vi "Read Configuration to gRPC.vi"(8 "error in (no error)":errorcluster, 11 "CIFPlugin in":refnum<class "CAN_Reader_CANsub_Plugin.lvclass">) -> (0 "error out":errorcluster, 2 "Configuration":T1={"Common"={"Period (s)"=0.001, "Offset (us)"=0, "Priority"=100, "Processor"=-2, "External Clock"={"ClockID"=0, "Clock Name"="", "Publish Clock"=FALSE, "Convert Data Timestamps"=FALSE, "Plugin Timing Source"=FALSE}}, "RX Interface"="CAN2", "Port Configuration"={"Mode"=enum."CAN FD", "Baud Rate"=500000, "Temination On"=TRUE, "Subordinate"=FALSE, "Echo TX"=FALSE, "FD Config"={"FD Baud Rate"=2000000, "ISO Mode"=TRUE, "BRS Enabled"=TRUE}}, "Timeout (ms)"=100, "Frames to read"=100, "Filter"={"Allow List (ID)"=[], "Deny List (ID)"=[]}} {"Filter"."Deny List (ID)" format="%.0x"; "Filter"."Allow List (ID)" format="%.0x"; "Port Configuration"."FD Config"."FD Baud Rate" format="%.0p"; "Port Configuration"."Baud Rate" format="%.0p"; "Common"."Period (s)" format="%#_13g"}, 3 "CIFPlugin out":refnum<class "CAN_Reader_CANsub_Plugin.lvclass">)   [LabVIEW 2021, in "CAN_Reader_CANsub_Plugin.lvclass"]
doc: "Updates to the configuration will not be automatically updated in the custom gRPC loop. To get the latest configuration the DVR used to pass configuration data from the core gRPC loop to the main loop can be read directly."
uses:
  CAN_Reader_CANsub_Plugin.lvclass
  CAN_Reader_CANsub_Plugin.lvclass/CAN_Reader_CANsub_Plugin.ctl
  <vilib>/CIF Foundation/CIF Core/CIFCore/Class/CIFCorePlugin.lvclass
  C:/Program Files/National Instruments/LabVIEW 2021/vi.lib/CIF Foundation/CIF Core/CIFCore/Class/CIFCorePlugin.lvclass
  D:/dev/Plugins/CAN_Reader_CANsub/Class/CAN_Reader_CANsub_Plugin.lvclass
  <vilib>/CIF Foundation/CIF Core/CIFCore/Common/Typedef/External Clock Config.ctl
  <vilib>/CIF Foundation/CIF Core/CIFCore/Common/CIFCoreCommon.lvlib
  <vilib>/CIF Foundation/CIF Core/CIFCore/Common/Typedef/Common Plugin Configuration.ctl
  Common/Typedef/Configuration.ctl
  Common/CAN_Reader_CANsub_Common.lvlib
  <vilib>/CIF Foundation/CIF CAN RW Core/typedef/CAN Mode.ctl
  <vilib>/CIF Foundation/CIF CAN RW Core/CAN_RW_CORE.lvclass
  <vilib>/CIF Foundation/CIF CAN RW Core/typedef/FD Config.ctl
  <vilib>/CIF Foundation/CIF CAN RW Core/typedef/CAN Port Configuration.ctl
  <vilib>/CIF Foundation/CIF CAN RW Core/typedef/CAN Filter.ctl
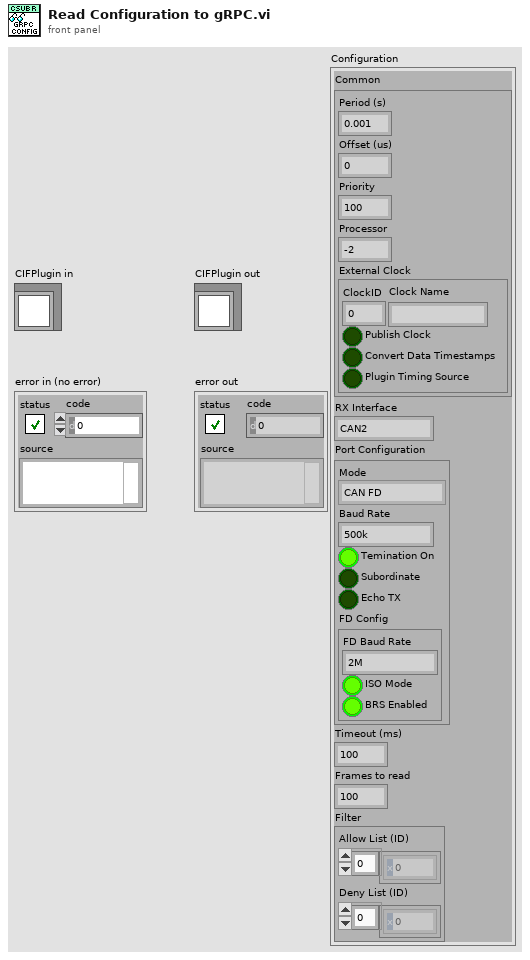
[diagram p1: front panel]
types:
  T1 = typedef "CAN_Reader_CANsub_Common.lvlib/Configuration.ctl" = cluster{"Common":T2, "RX Interface":string, "Port Configuration":T4, "Timeout (ms)":i32, "Frames to read":i32, "Filter":T7}
  T2 = typedef "CIFCoreCommon.lvlib/Common Plugin Configuration.ctl" = cluster{"Period (s)":dbl, "Offset (us)":i32, "Priority":i32, "Processor":i32, "External Clock":T3}
  T3 = typedef "CIFCoreCommon.lvlib/External Clock Config.ctl" = cluster{"ClockID":u8, "Clock Name":string, "Publish Clock":bool, "Convert Data Timestamps":bool, "Plugin Timing Source":bool}
  T4 = typedef "CAN_RW_CORE.lvclass/CAN Port Configuration.ctl" = cluster{"Mode":T5, "Baud Rate":u64, "Temination On":bool, "Subordinate":bool, "Echo TX":bool, "FD Config":T6}
  T5 = typedef "CAN_RW_CORE.lvclass/CAN Mode.ctl" = enum16{"CAN 2.0", "CAN FD"}
  T6 = typedef "CAN_RW_CORE.lvclass/FD Config.ctl" = cluster{"FD Baud Rate":u64, "ISO Mode":bool, "BRS Enabled":bool}
  T7 = typedef "CAN_RW_CORE.lvclass/CAN Filter.ctl" = cluster{"Allow List (ID)":u32[], "Deny List (ID)":u32[]}
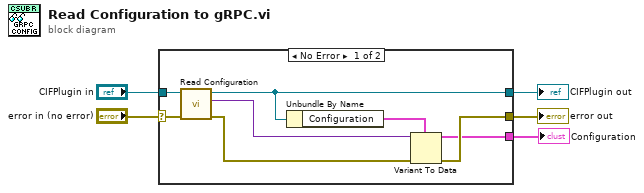
[diagram p0: block diagram]
diagram:
  n1 = case shown="No Error" "error in (no error)" {
    selector: "error in (no error)" -> [w12 w14]
    tunnel: "CIFPlugin in" -> [w13 w15]
    tunnel: [w7 w15] -> w2
    tunnel: [w8 w14] -> w4
    tunnel: [w6 _] -> w1
    frame No Error {
      n2 = call <vilib>:"Read Configuration.vi"("error in"=w12, "CIFCorePlugin in"=w13) -> ("error out"=w11:errorcluster, "Configuration Data"=w10:variant, "CIFCorePlugin out"=w7:refnum<class "CAN_Reader_CANsub_Plugin.lvclass">)  [unwired: 7 in]
      n3 = Unbundle By Name(w7) -> ("Configuration"=w9:T1)
      n4 = Variant To Data(error in=w11, type=w9, Variant=w10) -> (data=w6:T1, error out=w8:errorcluster)
    }
    frame Error {
    }
  }
  "error out" <- w4
  "CIFPlugin out" <- w2
  "Configuration" <- w1
